vi "Serial Port Write Simulator.vi"(0 "Port":u16, 1 "String":string) -> ()   [LabVIEW 2014]
uses:
  SimulatorGlobalOscilloscope.vi
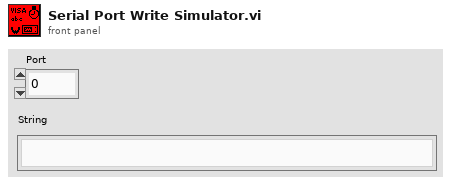
[diagram p1: front panel]
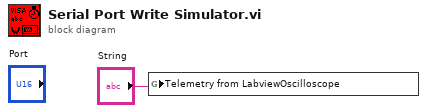
[diagram p0: block diagram]
diagram:
  n1 = global write "SimulatorGlobalOscilloscope.vi" "Telemetry from LabviewOscilloscope"("String") -> ()
